vi "get or create dataset from asset.vi"(10 "Datascope Name":string, 11 "asset":refnum<class "asset.lvclass">) -> (0 "error out":errorcluster, 2 "dataset":refnum<class "dataset.lvclass">, 3 "refreshed asset":refnum<class "asset.lvclass">)   [LabVIEW 2020, in "nominal core steps.lvlib"]
doc: "Locate a dataset on an asset, creating that dataset if not found.\n<b> </b> <b> </b>"
uses:
  nominal core steps.lvlib
  <vilib>/Nominal/Nominal IO Client/lv_src/asset/asset.lvclass
  <vilib>/Nominal/Nominal IO Client/lv_src/datasources/dataset/dataset.lvclass
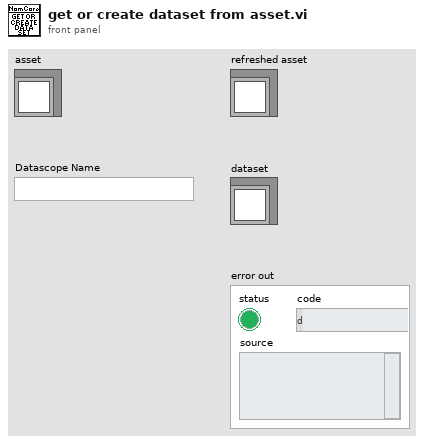
[diagram p1: front panel]
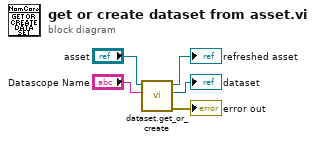
[diagram p0: block diagram]
diagram:
  n1 = call <vilib>:"dataset.get_or_create.vi"("Datascope Name"="Datascope Name", "asset in"="asset") -> ("error out"=→"error out":errorcluster, "dataset"=→"dataset":refnum<class "dataset.lvclass">, "asset out"=→"refreshed asset":refnum<class "asset.lvclass">)  [unwired: 7 in]
